vi "Configure Module.vi"(8 "error in (no error)":errorcluster, 10 "IOV ref in":variant, 11 "Module Template in":refnum<class "9402.lvclass">) -> (0 "error out":errorcluster, 2 "IOV ref out":variant, 3 "Module Template out":refnum<class "9402.lvclass">)   [LabVIEW 2020, in "Modules.lvlib" / "9402.lvclass"]
uses:
  9402.lvclass
  <resource>/objmgr/cRIO.rc
  SD Module/SD Module.lvclass
  C:/Users/nitest/Desktop/Git 2020/niveristand-scan-engine-module-libraries/Source/SD Module/SD Module.lvclass
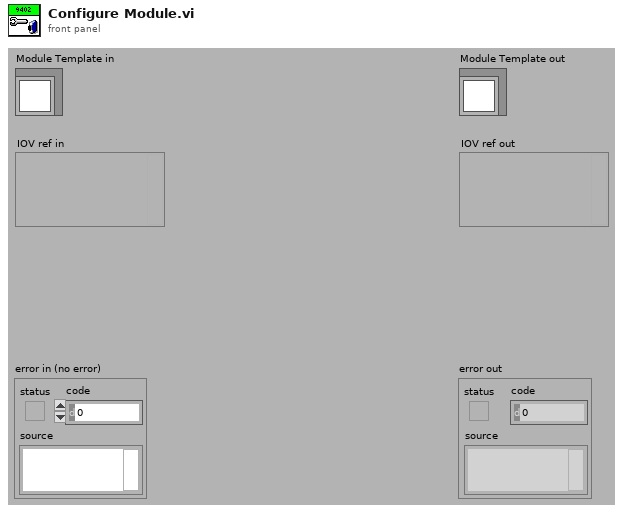
[diagram p1: front panel]
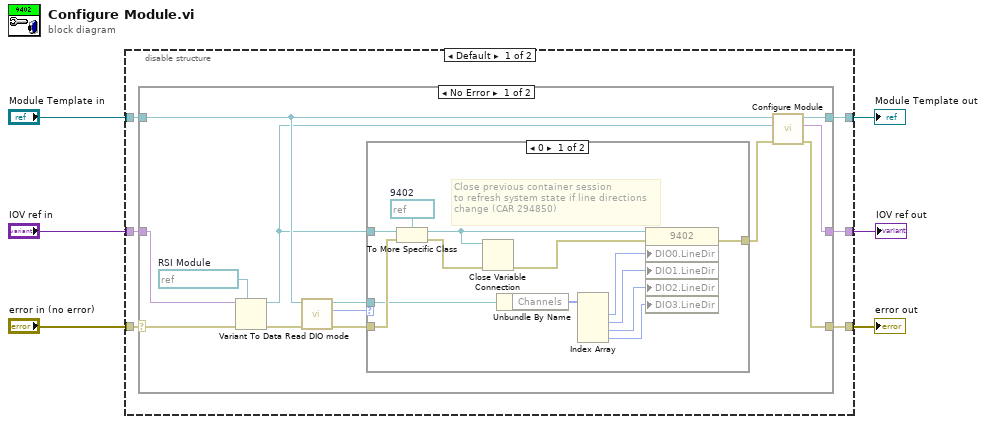
[diagram p0: block diagram]
diagram:
  n1 = disable-structure shown="Default" {
    disable-tunnel: "error in (no error)" -> [w12 w43]
    disable-tunnel: [w11 w43] -> w5
    disable-tunnel: "Module Template in" -> [w10 w45]
    disable-tunnel: [w9 w45] -> w3
    disable-tunnel: "IOV ref in" -> [w8 w44]
    disable-tunnel: [w7 w44] -> w1
    frame condition #0 {
      n2 = case shown="No Error" w12 {
        selector: w12 -> [w17 w42]
        tunnel: [w21 w42] -> w11
        tunnel: [w18 w41] -> w9
        tunnel: w10 -> [w19 w41]
        tunnel: w8 -> [w13 w40]
        tunnel: [w20 w40] -> w7
        frame No Error {
          w14 = refnum<k21> refnum  # RSI Module
          n3 = Variant To Data(error in=w17, type=w14, Variant=w13) -> (data=w15:refnum<k21>, error out=w16:errorcluster)
          n4 = call "Read DIO mode.vi"("error in (no error)"=w16, "SD Module in"=w19) -> ("error out"=w24:errorcluster, "DIO mode"=w23:u32, "SD Module out"=w25:refnum<class "9402.lvclass">)  [unwired: 7 in]
          n5 = case shown="0" w23 {
            tunnel: [w26 w39] -> w22
            tunnel: w15 -> [w37 _]
            tunnel: w25 -> [w27 _]
            tunnel: w24 -> [w28 w39]
            frame 0 {
              w38 = refnum<k21> refnum  # 9402
              # "Close previous container session\nto refresh system state if line directions\nchange (CAR 294850)"
              n6 = To More Specific Class(target class=w38, reference=w37, error in=w28) -> (specific class reference=w31:refnum<k21>, error out=w30:errorcluster)
              n7 = Close Variable Connection(8:w30, 11:w31) -> (0:w29:errorcluster)
              n8 = Unbundle By Name(w27) -> ("Channels"=w36:u32[])
              n9 = Index Array(array=w36) -> (element #1=w35:u32, element #2=w34:u32, element #3=w33:u32, element #4=w32:u32)  [unwired: 4 in]
              n10 = property class="9402"(reference=w31, error in=w29, "DIO0.LineDir"=w35, "DIO1.LineDir"=w34, "DIO2.LineDir"=w33, "DIO3.LineDir"=w32) -> (error out=w26:errorcluster)  [unwired: 1 out]
            }
            frame Default {
            }
          }
          n11 = call-parent "Configure Module.vi"("error in (no error)"=w22, "IOV ref in"=w15, "Module Template in"=w19) -> ("error out"=w21:errorcluster, "IOV ref out"=w20:variant, "Module Template out"=w18:refnum<class "9402.lvclass">)  [unwired: 6 in]
        }
        frame Error {
        }
      }
    }
    frame condition #1 (active) {
    }
  }
  "error out" <- w5
  "Module Template out" <- w3
  "IOV ref out" <- w1
